vi "关闭Helper Loop.vi"(0 "Display State In":T1 caption="显示状态输入", 9 "Container State":T3 caption="容器状态", 11 "error in (no error)":errorcluster caption="错误输入（无错误）") -> (4 "Display State Out":T1 caption="显示状态输出", 15 "error out":errorcluster caption="错误输出")   [LabVIEW 2025, in "XButton.lvlib" / "button3.xctl"]
uses:
  button3.xctl
  <vilib>/_xctls/Container State.ctl
  helper loop Events.ctl
  move event.ctl
  <vilib>/_xctls/XControlSupport.lvlib
panel:
  # "添加构成方法参数的输入控件及显示控件。连接至连线板。不要删除已连接至连线板的输入控件及显示控件。\n\n如需设置该方法的参数，右键单击项目树中的对应项并选择“配置方法...”。"
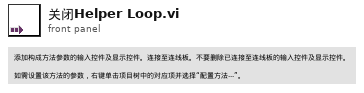
[diagram p1: front panel]
types:
  T1 = typedef "XButton.lvlib/button3.xctl/状态.ctl" = cluster{"Numeric":dbl, "调用方窗格颜色":u32, "按钮颜色":u32, "helper loop data":T2, "布尔文本":string, "字体颜色":u32, "字号":u32, "动效风格":enum16{"风格一", "风格二", "风格三", "风格四"}, "已隐藏不需要遮罩层":bool, "已初始化遮罩层位置":bool}
  T2 = typedef "XButton.lvlib/button3.xctl/helper loop Events.ctl" = cluster{"停止用户事件":refnum<user-event>, "修饰1move用户事件输出":refnum<user-event>, "修饰2move用户事件输出":refnum<user-event>}
  T3 = typedef "XControlSupport.lvlib/Container State.ctl" = cluster{"Indicator?":bool, "Run Mode?":bool, " Refnum":refnum<vi>}
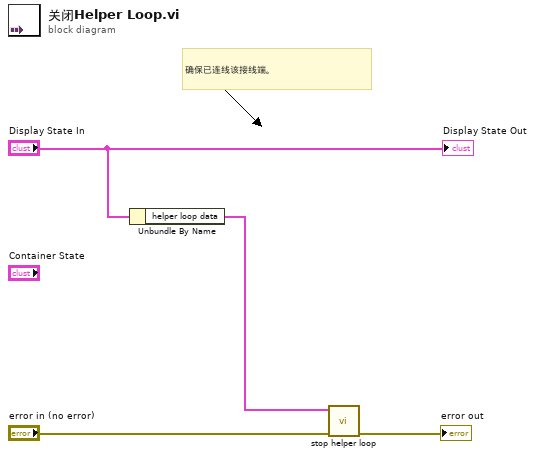
[diagram p0: block diagram]
diagram:
  # "确保已连线该接线端。"
  n1 = Unbundle By Name("Display State In") -> ("helper loop data"=w1:T2)
  n2 = call "stop helper loop.vi"("错误输入（无错误）"="error in (no error)", "helper loop data"=w1) -> ("错误输出"=→"error out":errorcluster)  [unwired: 9 in]
  "Display State Out" <- "Display State In"
